vi "clock_gettime.vi"(8 "error in (no error)":errorcluster, 11 "clock id (monotonic)":T1=enum."Monotonic") -> (0 "error out":errorcluster, 3 "timespec":cluster{"sec":u64, "nsec":u64})   [LabVIEW 2013, in "Linux RT Utilities.lvlib"]
doc: "Wrapper VI for glibc's clock_gettime() function."
uses:
  Linux RT Utilities.lvlib
  Controls/Public/C Enums/clockid_t.ctl
  <vilib>/Utility/error.llb/Error Cluster From Error Code.vi
  <vilib>/NI/NI Linux RT Errno/VIs/Public/Get LV Error Info from Errno.vi
  <vilib>/NI/NI Linux RT Errno/Linux Errno.lvlib
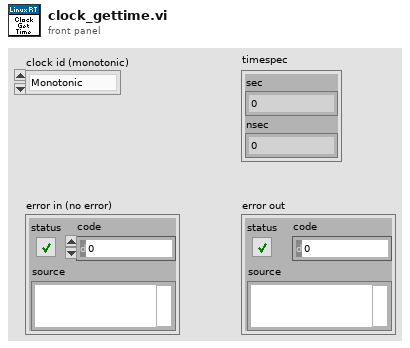
[diagram p1: front panel]
types:
  T1 = typedef "Linux RT Utilities.lvlib/clockid_t.ctl" = enum16{"Realtime", "Monotonic"}
  T2 = typedef "Linux Errno.lvlib/errno.ctl" = enum16{"NO ERROR", "EPERM", "ENOENT", "ESRCH", "EINTR", "EIO", "ENXIO", "E2BIG", "ENOEXEC", "EBADF", "ECHILD", "EAGAIN", "ENOMEM", "EACCES", "EFAULT", "ENOTBLK", "EBUSY", "EEXIST", "EXDEV", "ENODEV", "ENOTDIR", "EISDIR", "EINVAL", "ENFILE", "EMFILE", "ENOTTY", "ETXTBSY", "EFBIG", "ENOSPC", "ESPIPE", "EROFS", "EMLINK", "EPIPE", "EDOM", "ERANGE", "EDADLK", "ENAMETOOLONG", "ENOLCK", "ENOSYS", "ENOTEMPTY", "ELOOP", "EWOULDBLOCK", "ENOMSG", "EIDRM", "ECHRNG", "EL2NSYNC", "EL3HLT", "EL3RST", "ELNRNG", "EUNATCH", "ENOCSI", "EL2HLT", "EBADE", "EBADR", "EXFULL", "ENOANO", "EBADRQC", "EBADSLT", "EDEADLOCK", "EBFONT", "ENOSTR", "ENODATA", "ETIME", "ENOSR", "ENONET", "ENOPKG", "EREMOTE", "ENOLINK", "EADV", "ESRMNT", "ECOMM", "EPROTO", "EMULTIHOP", "EDOTDOT", "EBADMSG", "EOVERFLOW", "ENOTUNIQ", "EBADFD", "EREMCHG", "ELIBACC", "ELIBBAD", "ELIBSCN", "ELIBMAX", "ELIBEXEC", "ELISEQ", "ERESTART", "ESTRPIPE", "EUSERS", "ENOTSOCK", "EDESTADDRREQ", "EMSGSIZE", "EPROTOTYPE", "ENOPROTOOPT", "EPROTONOSUPPORT", "ESOCKTNOSUPPORT", "EOPNOTSUPP", "EPFNOSUPPORT", "EAFNOSUPPORT", "EADDRINUSE", "EADDRNOTAVAIL", "ENETDOWN", "ENETUNREACH", "ENETRESET", "ECONNABORTED", "ECONNRESET", "ENOBUFS", "EISCONN", "ENOTCONN", "ESHUTDOWN", "ETOOMANYREFS", "ETIMEDOUT", "ECONNREFUSED", "EHOSTDOWN", "EHOSTUNREACH", "EALREADY", "EINPROGRESS", "ESTALE", "EUCLEAN", "ENOTNAM", "ENAVAIL", "EISNAM", "EREMOTEIO", "EDQUOT", "ENOMEDIUM", "EMEDIUMTYPE", "ECANCELED", "ENOKEY", "EKEYEXPIRED", "EKEYREVOKED", "EKEYREJECTED", "EOWNERDEAD", "ENOTRECOVERABLE", "ERFKILL", "EHWPOISON", "UNDEFINED"}
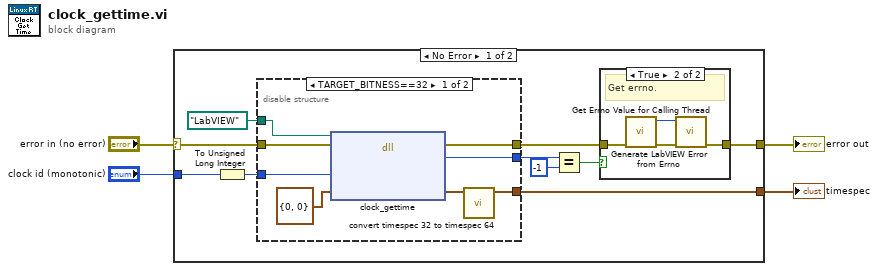
[diagram p0: block diagram]
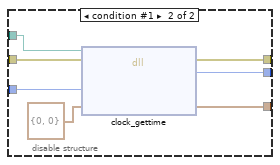
[diagram p3: hidden frame]
diagram:
  n1 = case shown="No Error" "error in (no error)" {
    selector: "error in (no error)" -> [w5 w35]
    tunnel: [w7 w35] -> w4
    tunnel: [w14 _] -> w1
    tunnel: "clock id (monotonic)" -> [w13 _]
    frame No Error {
      n2 = To Unsigned Long Integer(number=w13) -> (unsigned 32bit integer=w12:u32)
      n3 = disable-structure shown="TARGET_BITNESS==32" {
        disable-tunnel: w5 -> [w21 w34]
        disable-tunnel: w12 -> [w27 w33]
        disable-tunnel: [w24 w30] -> w14
        disable-tunnel: [w23 w32] -> w9
        disable-tunnel: [w22 w31] -> w11
        disable-tunnel: path "LabVIEW" ("Path") -> [w20 w28]
        frame condition #0 (active) {
          n4 = dll-call lib="lib/libc.so.6" fn="clock_gettime"(path in=w20, error in=w21, "clock_id"=w27, "timespec"=cluster{"sec":u32, "nsec":u32} {"sec"=0, "nsec"=0}) -> (error out=w23:errorcluster, "status"=w22:i32, "timespec"=w25:cluster{"sec":u32, "nsec":u32})  [unwired: 2 in, 1 out]
          n5 = call "convert timespec 32 to timespec 64.vi"("timespec 32"=w25) -> ("timespec 64"=w24:cluster{"sec":u64, "nsec":u64})  [unwired: 10 in]
        }
        frame condition #1 {
          n6 = dll-call lib="lib/libc.so.6" fn="clock_gettime"(path in=w28, error in=w34, "clock_id"=w33, "timespec"=cluster{"sec":u64, "nsec":u64} {"sec"=0, "nsec"=0}) -> (error out=w32:errorcluster, "status"=w31:i32, "timespec"=w30:cluster{"sec":u64, "nsec":u64})  [unwired: 2 in, 1 out]
        }
      }
      n7 = Equal?(x=w11, y=-1) -> (x = y?=w8:bool)
      n8 = case shown="True" w8 {
        tunnel: w9 -> [w15 w19]
        tunnel: [w15 w16] -> w7
        frame False {
          # "No error."
        }
        frame True {
          # "Get errno."
          n9 = call <vilib>:"Get Errno Value for Calling Thread.vi"("error in (no error)"=w19) -> ("error out"=w18:errorcluster, "errno"=w17:T2)  [unwired: 9 in]
          n10 = call <vilib>:"Generate LabVIEW Error from Errno.vi"("error in (no error)"=w18, "errno"=w17) -> ("error out"=w16:errorcluster)  [unwired: 9 in]
        }
      }
    }
    frame Error {
    }
  }
  "error out" <- w4
  "timespec" <- w1
